vi "FuncVI-FilePathToArray.vi"(5 "InstanceRef":T2, 9 "arg list":T1[](array[typedef]) {"num" format="%.2f"}) -> (0 "error out":bool, 3 "result":T1 {"num" format="%.2f"})   [LabVIEW 2021]
doc: "::: CalcExpress Toolkit :::\nCopyright (c) 2000-2026 Konstantin Shifershteyn. All rights reserved."
uses:
  cetypes.llb/CalcExpress Function Argument Info.ctl
  cetypes.llb/CalcExpress Instance RefNum.ctl
panel:
  in  "max arg num":i32=2
  in  "min arg num":i32=1
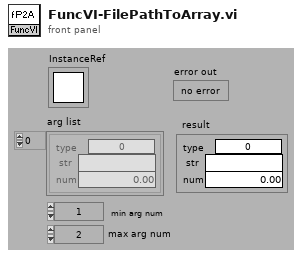
[diagram p1: front panel]
types:
  T1 = typedef "CalcExpress Function Argument Info.ctl" = cluster{"type":u32, "str":string, "num":dbl}
  T2 = typedef "CalcExpress Instance RefNum.ctl" = refnum<k1>
  T3 = cluster{"index":i32, "data type":enum32{"String", "DBL Number", "identifier", "1D Array of DBL", "2D Array of DBL", "CDB Number", "1D Array of CDB", "2D Array of CDB", "1D Array of String", "2D Array of String", "Unknown data type"}, "default num":dbl, "default str":string}[]
  T4 = enum32{"String", "DBL Number", "identifier", "1D Array of DBL", "2D Array of DBL", "CDB Number", "1D Array of CDB", "2D Array of CDB", "1D Array of String", "2D Array of String", "Unknown data type"}
  T5 = cluster{"type: use this constant to specify a predefined type code":enum32{"String", "DBL Number", "identifier", "1D Array of DBL", "2D Array of DBL", "CDB Number", "1D Array of CDB", "2D Array of CDB", "1D Array of String", "2D Array of String", "Unknown data type"}, "data string":string, dbl}
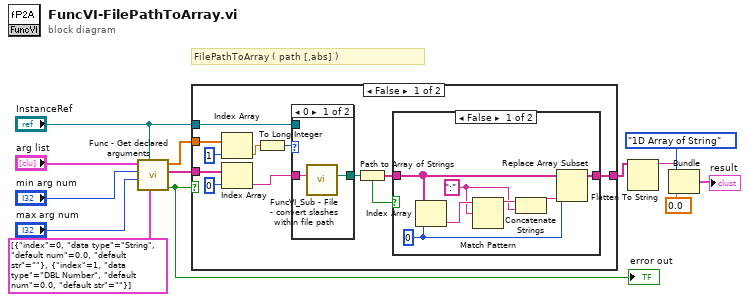
[diagram p0: block diagram]
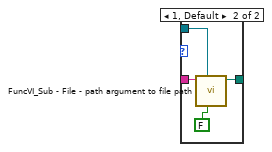
[diagram p3: hidden frame]
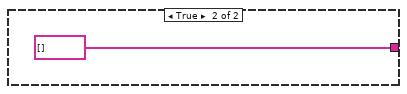
[diagram p4: hidden frame]
diagram:
  # "FilePathToArray ( path [,abs] )"
  n1 = call "Func - Get declared arguments.vi"("arg descriptors"=T3 [{"index"=0, "data type"=enum."String", "default num"=0.0, "default str"=""}, {"index"=1, "data type"=enum."DBL Number", "default num"=0.0, "default str"=""}], "InstanceRef"="InstanceRef", "max arg num"="max arg num", "min arg num"="min arg num", "arg list"="arg list") -> ("error out"=w5:bool, "str list"=w9:string[], "num list"=w3:dbl[])  [unwired: 3 in, 1 out]
  "error out" <- w5
  n2 = case shown="False" w5 {
    tunnel: "InstanceRef" -> [w22 _]
    tunnel: w9 -> [w23 _]
    tunnel: [w14 string[] [] ("array of strings")] -> w7
    tunnel: w3 -> [w19 _]
    frame False {
      n3 = Index Array(array=w19, index=1) -> (element=w18:dbl)
      n4 = Index Array(array=w23, index=0) -> (element=w24:string)
      n5 = To Long Integer(number=w18) -> (32bit integer=w17:i32)
      n6 = case shown="0" w17 {
        tunnel: w24 -> [w34 w39]
        tunnel: w22 -> [_ w38]
        tunnel: [w35 w37] -> w21
        frame 0 {
          n7 = call "FuncVI_Sub - File - convert slashes within file path.vi"("str: path"=w34) -> ("path out"=w35:path)  [unwired: 3 in, 1 out]
        }
        frame 1, Default {
          n8 = call "FuncVI_Sub - File - path argument to file path.vi"("allow dialog"=FALSE, "InstanceRef"=w38, "arg: file path"=w39) -> ("file path"=w37:path)  [unwired: 6 in, 2 out]
        }
      }
      n9 = Path to Array of Strings(0:w21) -> (1:w16:bool, 2:w15:string[])
      n10 = case shown="False" w16 {
        tunnel: w15 -> [w27 w33]
        tunnel: [w26 w33] -> w14
        frame False {
          w30 = ":" ("regular expression")
          w28 = 0
          n11 = Index Array(array=w27, index=w28) -> (element=w32:string)
          n12 = Match Pattern(string=w32, regular expression=w30) -> (before substring=w31:string)  [unwired: 1 in, 3 out]
          n13 = Concatenate Strings(w31, w30) -> (w29:string)
          n14 = Replace Array Subset(array=w27, new element=w29, index=w28) -> (w26:string[])
        }
        frame True {
        }
      }
    }
    frame True {
    }
  }
  n15 = Flatten To String(anything=w7) -> (data string=w6:string)  [unwired: 3 in, 2 out]
  n16 = Bundle("type: use this constant to specify a predefined type code"=T4."1D Array of String", "data string"=w6, 0.0) -> (→"result":T5)  [unwired: 1 in]
